vi "CSV String to Array.vi"(8 "error in":errorcluster, 10 "CSV Spreadsheet String":string) -> (0 "error out":errorcluster, 2 "Array":string[][](array[string]))   [LabVIEW 2020]
uses:
  source/library/openg_string.lvlib
panel:
  # "CSV String to Array.vi\n\nConverts a Comma Seperated Values (CSV) spreadsheet string to an array.\n\nPlease visit http://www.OpenG.org to learn about the\nOpen Source LabVIEW software movement.\n\nNOTICE -- YOU MUST LEAVE THIS NOTICE IN PLACE.  PER THE TERMS OF THE LICENSE BELOW, YOU MAY SUBLICENSE THIS SOFTWARE \nIN ANY WAY THAT DOES NOT CONFLICT WITH THIS LICENSE.\n\n### BSD License (http://www.opensource.org/licenses/bsd-license.php) Begin ###\n \nCopyright (c) 2006, James Kring, Inc. (Author: Jim Kring <jim.kring@jameskring.com>)\n\nAll rights reserved.\n\nRedistribution and use in source and binary forms, with or without modification, are permitted provided that the following conditions are met:\n\n    * Redistributions of source code must retain the above copyright notice, this list of conditions and the following disclaimer.\n    * Redistributions in binary form must reproduce the above copyright notice, this list of conditions and the following disclaimer in the \n       documentation and/or other materials provided with the distribution.\n    * Neither the name of SciWare, James Kring, Inc., nor the names of its contributors may be used to endorse or promote products derived \n       from this software without specific prior written permission.\n\nTHIS SOFTWARE IS PROVIDED BY THE COPYRIGHT HOLDERS AND CONTRIBUTORS \"AS IS\" AND ANY EXPRESS OR IMPLIED WARRANTIES, \nINCLUDING, BUT NOT LIMITED TO, THE IMPLIED WARRANTIES OF MERCHANTABILITY AND FITNESS FOR A PARTICULAR PURPOSE ARE \nDISCLAIMED. IN NO EVENT SHALL THE COPYRIGHT OWNER OR CONTRIBUTORS BE LIABLE FOR ANY DIRECT, INDIRECT, INCIDENTAL,\n SPECIAL, EXEMPLARY, OR CONSEQUENTIAL DAMAGES (INCLUDING, BUT NOT LIMITED TO, PROCUREMENT OF SUBSTITUTE GOODS OR \nSERVICES; LOSS OF USE, DATA, OR PROFITS; OR BUSINESS INTERRUPTION) HOWEVER CAUSED AND ON ANY THEORY OF LIABILITY, \nWHETHER IN CONTRACT, STRICT LIABILITY, OR TORT (INCLUDING NEGLIGENCE OR OTHERWISE) ARISING IN ANY WAY OUT OF THE USE \nOF THIS SOFTWARE, EVEN IF ADVISED OF THE POSSIBILITY OF SUCH DAMAGE.\n\n### BSD License End ###"
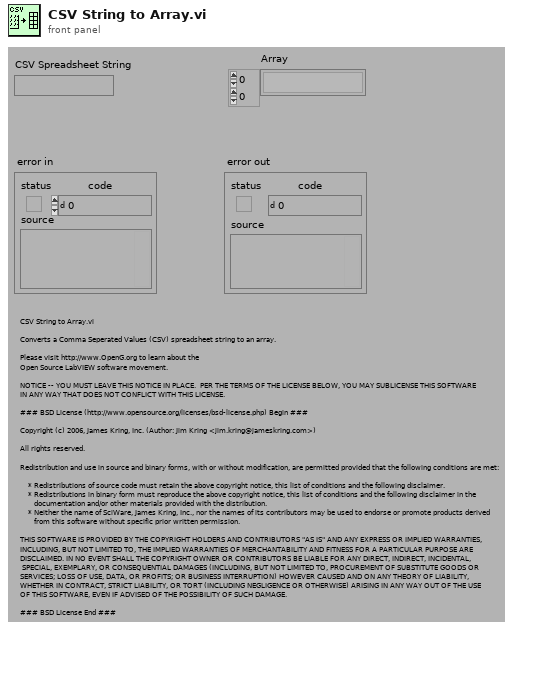
[diagram p1: front panel]
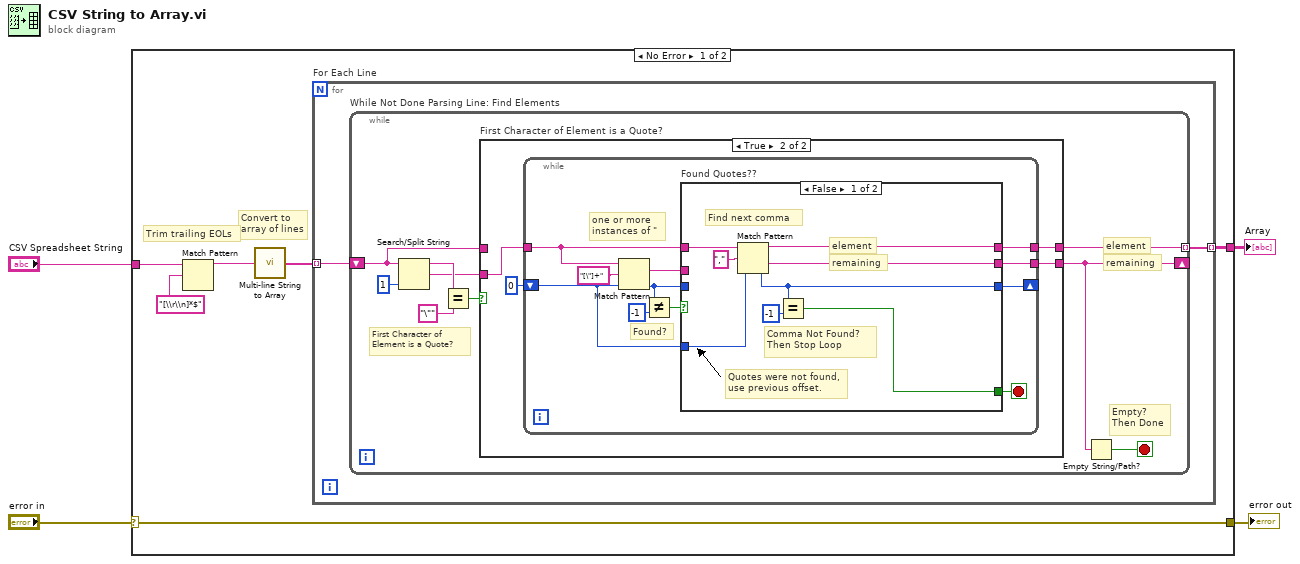
[diagram p0: block diagram]
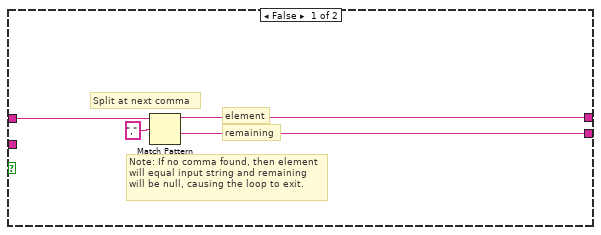
[diagram p2: hidden frame]
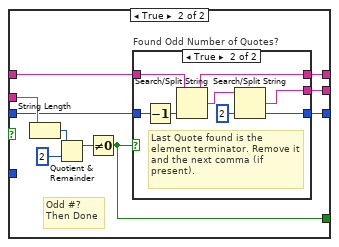
[diagram p3: hidden frame]
diagram:
  n1 = case shown="No Error" "error in" {
    selector: "error in" -> [w5 w69]
    tunnel: [w9 _] -> w1
    tunnel: "CSV Spreadsheet String" -> [w6 _]
    tunnel: [w5 w69] -> w4
    frame No Error {
      # "Convert to array of lines"
      # "Trim trailing EOLs"
      n2 = Match Pattern(string=w6, regular expression="[\\r\\n]*$") -> (before substring=w7:string)  [unwired: 1 in, 3 out]
      n3 = call "Multi-line String to Array.vi"("string"=w7) -> ("lines"=w10:string[])
      n4 = for "For Each Line" {
        tunnel: w10 -> [w12] mode=indexing
        tunnel: [w11] -> w9 mode=indexing
        n5 = while "While Not Done Parsing Line: Find Elements" {
          tunnel: [w15] -> w11 mode=indexing
          shift-right: [w14] -> _
          shift-left: w12 -> [w16]
          stop <- w13 stop-if-true
          # "First Character of Element is a Quote?"
          # "remaining"
          # "element"
          # "Empty?\nThen Done"
          n6 = Search/Split String(string=w16, offset (0)=1) -> (substring before match=w19:string, match + rest of string=w17:string)  [unwired: 1 in, 1 out]
          n7 = Equal?(x=w19, y="\"" ("regular expression")) -> (x = y?=w18:bool)
          n8 = case "First Character of Element is a Quote?" shown="True" w18 {
            tunnel: w17 -> [_ w29]
            tunnel: w16 -> [w24 _]
            tunnel: [w22 w26] -> w15
            tunnel: [w23 w27] -> w14
            frame False {
              # "remaining"
              # "element"
              # "Note: If no comma found, then element will equal input string and remaining will be null, causing the loop to exit."
              # "Split at next comma"
              n9 = Match Pattern(string=w24, regular expression=",") -> (before substring=w22:string, after substring=w23:string)  [unwired: 1 in, 2 out]
            }
            frame True {
              n10 = while {
                tunnel: w29 -> [w38]
                shift-right: [w36] -> _
                shift-left: 0 ("offset past match") -> [w31]
                tunnel: [w37] -> w26
                tunnel: [w30] -> w27
                stop <- w35 stop-if-true
                # "Found?"
                # "one or more instances of \""
                n11 = Match Pattern(string=w38, regular expression="[\"]+", offset (0)=w31) -> (match substring=w39:string, offset past match=w34:i32)  [unwired: 2 out]
                n12 = Not Equal?(x=w34, y=-1) -> (x != y?=w32:bool)
                n13 = case "Found Quotes??" shown="False" w32 {
                  tunnel: w39 -> [_ w58]
                  tunnel: w38 -> [w47 w54]
                  tunnel: w34 -> [_ w53]
                  tunnel: [w45 w52] -> w37
                  tunnel: [w42 w51] -> w36
                  tunnel: [w41 w50] -> w35
                  tunnel: w31 -> [w46 _]
                  tunnel: [w44 w49] -> w30
                  frame False {
                    # "Find next comma"
                    # "Quotes were not found, use previous offset."
                    # "remaining"
                    # "element"
                    # "Comma Not Found?\nThen Stop Loop"
                    n14 = Match Pattern(string=w47, regular expression=",", offset (0)=w46) -> (before substring=w45:string, after substring=w44:string, offset past match=w42:i32)  [unwired: 1 out]
                    n15 = Equal?(x=w42, y=-1) -> (x = y?=w41:bool)
                  }
                  frame True {
                    # "Odd #?\nThen Done"
                    n16 = String Length(string=w58) -> (length=w57:i32)
                    n17 = Quotient & Remainder(x=w57, y=2) -> (x-y*floor(x/y)=w55:i32)  [unwired: 1 out]
                    n18 = Not Equal To 0?(x=w55) -> (x != 0?=w50:bool)
                    n19 = case "Found Odd Number of Quotes?" shown="True" w50 {
                      tunnel: w54 -> [w59 w67]
                      tunnel: w53 -> [w60 w68]
                      tunnel: [w59 w65] -> w52
                      tunnel: [w60 w64] -> w51
                      tunnel: [_ w61] -> w49
                      frame False {
                      }
                      frame True {
                        # "Last Quote found is the element terminator. Remove it and the next comma (if present)."
                        n20 = Decrement(x=w68) -> (x-1=w66:i32)
                        n21 = Search/Split String(string=w67, offset (0)=w66) -> (substring before match=w65:string, match + rest of string=w63:string)  [unwired: 1 in, 1 out]
                        n22 = Search/Split String(string=w63, offset (0)=2) -> (match + rest of string=w61:string, offset of match=w64:i32)  [unwired: 1 in, 1 out]
                      }
                    }
                  }
                }
              }
            }
          }
          n23 = Empty String/Path?(string/path=w14) -> (empty?=w13:bool)
        }
      }
    }
    frame Error {
    }
  }
  "error out" <- w4
  "Array" <- w1
